vi "Remove Permissions.vi"(8 "error in (no error)":errorcluster, 10 "Label":string, 11 "SQS in":refnum<class "Queue.lvclass">) -> (0 "error out":errorcluster, 3 "SQS out":refnum<class "Queue.lvclass">)   [LabVIEW 2015, in "NI_AWS_SQS.lvlib" / "Queue.lvclass"]
doc: "Revokes any permissions in the queue policy that matches the specified Label parameter. Only the owner of the queue can remove permissions."
uses:
  Queue.lvclass
  Core/HTTP Request/Name Value Pair.ctl
  Core/HTTP Request/Request Options.ctl
  Core/HTTP Request/Region handling.ctl
  Core/HTTP Request/URL formatting.ctl
  Queue.lvclass/Queue.ctl
  Read Account Number.vi
  Read Name.vi
  Core/HTTP Request/HTTP Request.lvclass
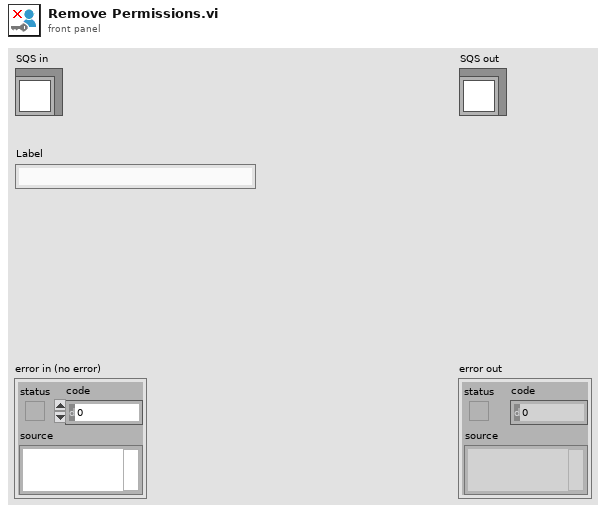
[diagram p1: front panel]
types:
  T1 = typedef "NI_AWS_Core.lvlib/HTTP Request.lvclass/Name Value Pair.ctl" = cluster{"name":string, "value":string}
  T2 = typedef "NI_AWS_Core.lvlib/HTTP Request.lvclass/Request Options.ctl" = cluster{"request headers":T1[], "request parameters":T1[], "request body":string, "region handling":T3, "URL formatting":T4}
  T3 = typedef "NI_AWS_Core.lvlib/HTTP Request.lvclass/Region handling.ctl" = enum16{"use region everywhere", "use region (authentication only)", "use region (URL only)", "ignore region everwhere"}
  T4 = typedef "NI_AWS_Core.lvlib/HTTP Request.lvclass/URL formatting.ctl" = enum16{"region-", "region."}
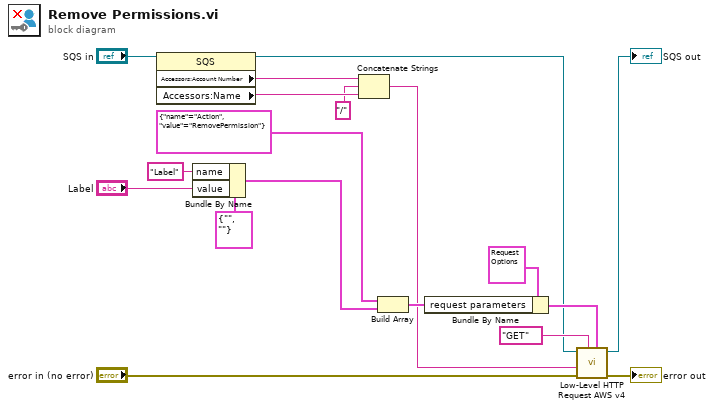
[diagram p0: block diagram]
diagram:
  n1 = property class="SQS"(reference="SQS in") -> (reference out=w1:refnum<class "Queue.lvclass">, "Accessors:Account Number"=w16:string, "Accessors:Name"=w15:string)  [unwired: 1 in, 1 out]
  n2 = Bundle By Name(cluster=T1 {"name"="", "value"=""} ("element"), "name"="Label", "value"="Label") -> (w7:T1)
  n3 = Concatenate Strings(w16, "/", w15) -> (w10:string)
  n4 = Build Array(T1 {"name"="Action", "value"="RemovePermission"} ("Cluster"), w7) -> (w17:T1[])
  n5 = Bundle By Name(cluster=T2 {"request headers"=[], "request parameters"=[{"name"="Action", "value"="ListQueues"}], "request body"="", "region handling"=enum."use region everywhere", "URL formatting"=enum."region."} ("Request Options"), "request parameters"=w17) -> (w3:T2)
  n6 = call "Low-Level HTTP Request AWS v4.vi"("Request Options"=w3, "HTTP-Verb"="GET", "error in (no error)"="error in (no error)", "URL Suffix"=w10, "AWS Core in"=w1) -> ("error out"=→"error out":errorcluster, "AWS Core out"=→"SQS out":refnum<class "Queue.lvclass">)  [unwired: 3 in, 2 out]
